vi "Post-Install Custom Action.vi"(10 "Variant":variant) -> (0 "error out":errorcluster)   [LabVIEW 2021]
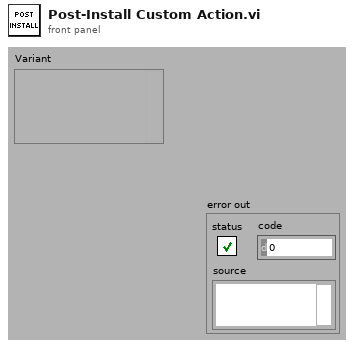
[diagram p1: front panel]
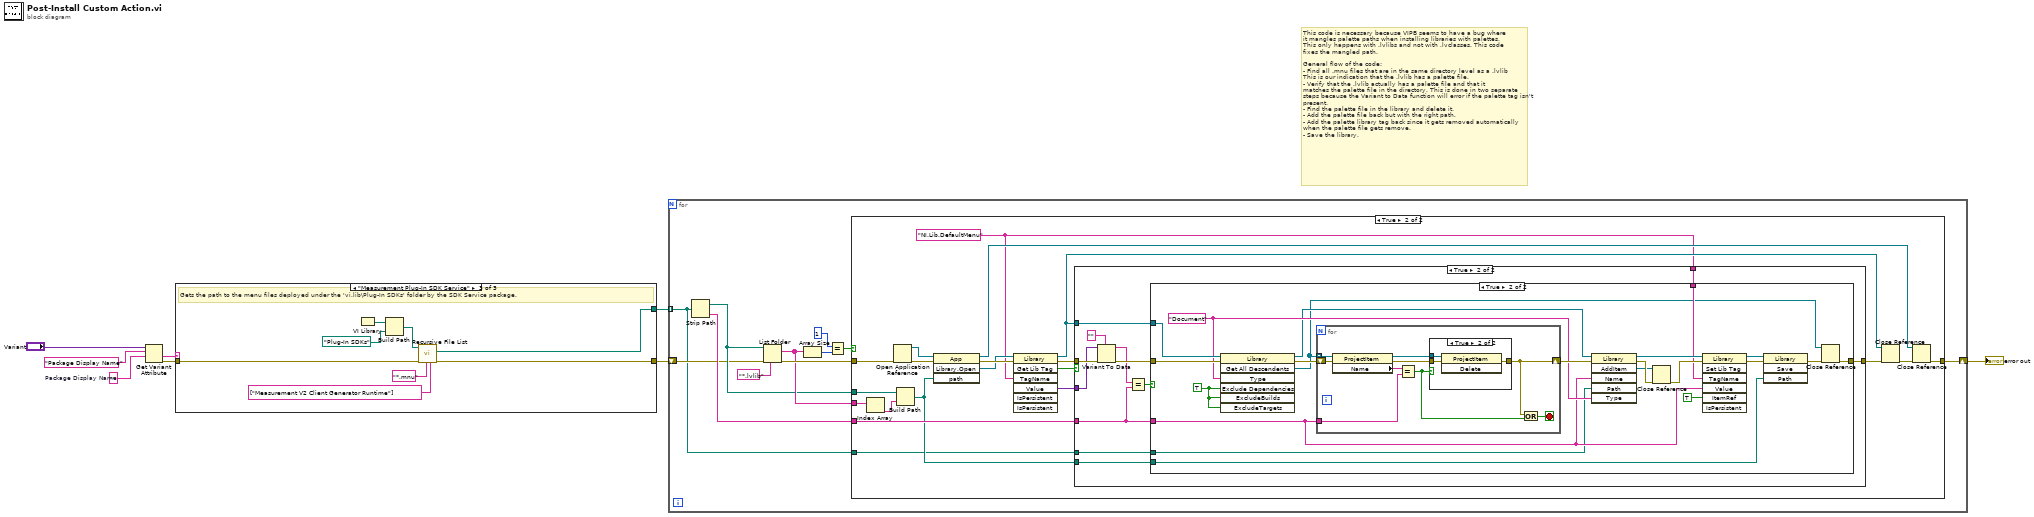
[diagram p0: block diagram]
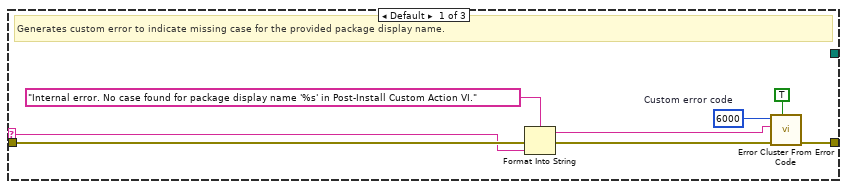
[diagram p6: hidden frame]
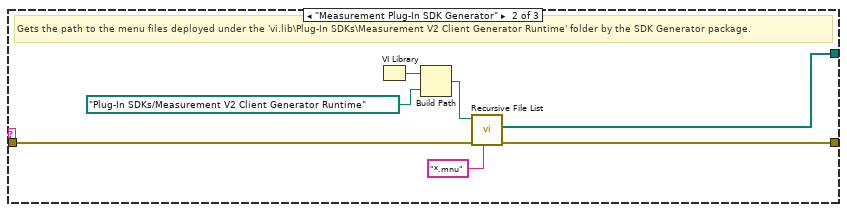
[diagram p7: hidden frame]
diagram:
  w7 = ""  # Package Display Name
  # "This code is necessary because VIPB seems to have a bug where\nit mangles palette paths when installing libraries with palettes.\nThis only happens with .lvlibs and not with .lvclasses. This code\nfixes the mangled path.\n\nGeneral flow of the code:\n- Find all .mnu files that are in the same directory level as a .lvlib\nThis is our indication that the .lvlib has a palette file.\n- Verify that the .lvlib actually has a palette file and that it\nmatches the palette file in the directory. This is done in two separate\nsteps because the Variant to Data function will error if the palette tag isn't\npresent.\n- Find the palette file in the library and delete it.\n- Add the palette file back but with the right path.\n- Add the palette library tag back since it gets removed automatically\nwhen the palette file gets remove.\n- Save the library."
  n1 = Get Variant Attribute(Variant="Variant", name="Package Display Name", default value (empty Variant)=w7) -> (value=w2:string, error out=w1:errorcluster)  [unwired: 1 in, 2 out]
  n2 = case shown="\"Measurement Plug-In SDK Service\"" w2 {
    selector: w2 -> [w13 _ _]
    tunnel: [_ w18 w29] -> w3
    tunnel: [w16 w19 w30] -> w4
    tunnel: w1 -> [w14 w17 w28]
    frame Default {
      w11 = 6000  # Custom error code
      # "Generates custom error to indicate missing case for the provided package display name."
      n3 = Format Into String(format string="Internal error. No case found for package display name '%s' in Post-Install Custom Action VI.", error in=w14, w13) -> (resulting string=w12:string, error out=w15:errorcluster)  [unwired: 1 in]
      n4 = call <vilib>:"Error Cluster From Error Code.vi"("show call chain? (False)"=TRUE, "error in (no error)"=w15, "error message (\"\")"=w12, "error code (0)"=w11) -> ("error out"=w16:errorcluster)  [unwired: 5 in]
    }
    frame "Measurement Plug-In SDK Generator" {
      # "Gets the path to the menu files deployed under the 'vi.lib\\Plug-In SDKs\\Measurement V2 Client Generator Runtime' folder by the SDK Generator package."
      n5 = VI Library() -> (path=w22:path)
      n6 = Build Path(base path=w22, name or relative path=path "Plug-In SDKs/Measurement V2 Client Generator Runtime") -> (appended path=w23:path)
      n7 = call <vilib>:"Recursive File List.vi"("pattern"="*.mnu", "error in (no error)"=w17, "Folder Path"=w23) -> ("error out"=w19:errorcluster, "All Files in Dir"=w18:path[])  [unwired: 4 in, 3 out]
    }
    frame "Measurement Plug-In SDK Service" {
      # "Gets the path to the menu files deployed under the 'vi.lib\\Plug-In SDKs' folder by the SDK Service package."
      n8 = VI Library() -> (path=w27:path)
      n9 = Build Path(base path=w27, name or relative path=path "Plug-In SDKs") -> (appended path=w31:path)
      n10 = call <vilib>:"Recursive File List.vi"("Folders to Exclude"=string[] ["Measurement V2 Client Generator Runtime"], "pattern"="*.mnu", "error in (no error)"=w28, "Folder Path"=w31) -> ("error out"=w30:errorcluster, "All Files in Dir"=w29:path[])  [unwired: 3 in, 3 out]
    }
  }
  n11 = for {
    shift-right: [w34] -> w6
    shift-left: w4 -> [w33]
    tunnel: w3 -> [w32] mode=indexing
    n12 = Strip Path(path=w32) -> (stripped path=w36:path, name=w40:string)
    n13 = List Folder(path=w36, pattern="*.lvlib", error in=w33) -> (filenames=w38:string[], error out=w39:errorcluster)  [unwired: 1 in, 2 out]
    n14 = Array Size(array=w38) -> (size(s)=w42:i32)
    n15 = Equal?(x=1, y=w42) -> (x = y?=w41:bool)
    n16 = case shown="True" w41 {
      tunnel: w39 -> [w43 w60]
      tunnel: w38 -> [_ w63]
      tunnel: w40 -> [_ w55]
      tunnel: w36 -> [_ w51]
      tunnel: [w43 w45] -> w34
      tunnel: w32 -> [_ w44]
      frame False {
      }
      frame True {
        w47 = "NI.Lib.DefaultMenu" ("Tag Name")
        n17 = Index Array(array=w63) -> (element=w50:string)  [unwired: 1 in]
        n18 = Open Application Reference(8:w60) -> (0:w62:errorcluster, 3:w61:refnum<vi>)  [unwired: 3 in]
        n19 = Build Path(base path=w51, name or relative path=w50) -> (appended path=w49:path)
        n20 = invoke class="App" method="Library.Open"(reference=w61, error in=w62, "path"=w49) -> (reference out=w52:refnum<vi>, error out=w59:errorcluster, "Open Library"=w56:refnum<vi>)  [unwired: 1 in, 1 out]
        n21 = invoke class="Library" method="Get Lib Tag"(reference=w56, error in=w59, "TagName"=w47) -> (reference out=w53:refnum<vi>, error out=w57:errorcluster, "GetTag"=w48:bool, "Value"=w58:variant)  [unwired: 4 in, 3 out]
        n22 = case shown="True" w48 {
          tunnel: w58 -> [_ w72]
          tunnel: w57 -> [w64 w73]
          tunnel: [w64 w76] -> w54
          tunnel: w53 -> [_ w75]
          tunnel: w49 -> [_ w74]
          tunnel: w55 -> [_ w68]
          tunnel: w47 -> [_ w66]
          tunnel: w44 -> [_ w65]
          frame False {
          }
          frame True {
            n23 = Variant To Data(error in=w73, type="", Variant=w72) -> (data=w69:string, error out=w71:errorcluster)
            n24 = Equal?(x=w69, y=w68) -> (x = y?=w67:bool)
            n25 = case shown="True" w67 {
              tunnel: [w77 w87] -> w76
              tunnel: w75 -> [_ w98]
              tunnel: w74 -> [_ w93]
              tunnel: w71 -> [w77 w92]
              tunnel: w68 -> [_ w79]
              tunnel: w66 -> [_ w84]
              tunnel: w65 -> [_ w78]
              frame False {
              }
              frame True {
                w86 = "Document" ("Type")
                w82 = TRUE ("ExcludeDependencies")
                n26 = invoke class="Library" method="Get All Descendents"(reference=w98, error in=w92, "Type"=w86, "Exclude Dependencies"=w82, "ExcludeBuilds"=w82, "ExcludeTargets"=w82) -> (reference out=w81:refnum<vi>, error out=w97:errorcluster, "All Descendents"=w80:refnum<vi>[])  [unwired: 1 in, 4 out]
                n27 = for {
                  tunnel: w80 -> [w107] mode=indexing
                  shift-right: [w101] -> w96
                  shift-left: w97 -> [w103]
                  tunnel: w79 -> [w102]
                  stop <- w99 stop-if-true
                  n28 = property class="ProjectItem"(reference=w107, error in=w103) -> (reference out=w105:refnum<vi>, error out=w104:errorcluster, "Name"=w106:string)
                  n29 = Equal?(x=w106, y=w102) -> (x = y?=w100:bool)
                  n30 = case shown="True" w100 {
                    tunnel: w105 -> [_ w111]
                    tunnel: w104 -> [w108 w109]
                    tunnel: [w108 w110] -> w101
                    frame False {
                    }
                    frame True {
                      n31 = invoke class="ProjectItem" method="Delete"(reference=w111, error in=w109) -> (error out=w110:errorcluster)  [unwired: 1 in, 2 out]
                    }
                  }
                  n32 = Or(x=w101, y=w100) -> (x .or. y?=w99:bool)
                }
                n33 = invoke class="Library" method="AddItem"(reference=w81, error in=w96, "Name"=w79, "Path"=w78, "Type"=w86) -> (reference out=w85:refnum<vi>, error out=w90:errorcluster, "AddItem"=w89:refnum<vi>)  [unwired: 1 in, 3 out]
                n34 = Close Reference(reference=w89, error in (no error)=w90) -> (error out=w88:errorcluster)
                n35 = invoke class="Library" method="Set Lib Tag"(reference=w85, error in=w88, "TagName"=w84, "Value"=w79, "ItemRef"=TRUE ("Is Persistent")) -> (reference out=w95:refnum<vi>, error out=w94:errorcluster)  [unwired: 2 in, 5 out]
                n36 = invoke class="Library" method="Save"(reference=w95, error in=w94, "Path"=w93) -> (error out=w91:errorcluster)  [unwired: 1 in, 3 out]
                n37 = Close Reference(reference=w80, error in (no error)=w91) -> (error out=w87:errorcluster)
              }
            }
          }
        }
        n38 = Close Reference(reference=w53, error in (no error)=w54) -> (error out=w46:errorcluster)
        n39 = Close Reference(reference=w52, error in (no error)=w46) -> (error out=w45:errorcluster)
      }
    }
  }
  "error out" <- w6
